vi "Initialization VI.vi"(8 "error in (no error)":errorcluster, 10 "Custom XML":string, 11 "Device Item Ref in":T1 format="%.0x") -> (0 "error out":errorcluster, 3 "Device Item Ref out":T1 format="%.0x")   [LabVIEW 2020, in "FPGA Addon System Explorer.lvlib"]
uses:
  FPGA Addon System Explorer.lvlib
  <vilib>/NI VeriStand/Custom Device API/Custom Device Item Ref.ctl
  Addon Shared/Types/FG Action.ctl
  Addon Shared/Types/FPGA Settings.ctl
  Addon Shared/SubVIs/Constants.vi
  <vilib>/NI VeriStand/Custom Device API/NI VeriStand - Get Item Property.vi
  <vilib>/NI VeriStand/Custom Device API/Get Item Property (Path).vi
  <vilib>/NI VeriStand/Custom Device API/Get Item Property (String).vi
  <vilib>/NI VeriStand/Custom Device API/Get Item Property (Boolean).vi
  <vilib>/NI VeriStand/Custom Device API/NI VeriStand - Set Item Property.vi
  <vilib>/NI VeriStand/Custom Device API/Set Item Property (Path).vi
  <vilib>/NI VeriStand/Custom Device API/Set Item Property (String).vi
  <vilib>/NI VeriStand/Custom Device API/Set Item Property (Boolean).vi
  <vilib>/NI/NI VeriStand Custom Device Import and Export Tool/ImportExport.lvlib
  Addon Shared/FPGA Addon Shared.lvlib
  <vilib>/NI VeriStand/Custom Device API/Custom Device API.lvlib
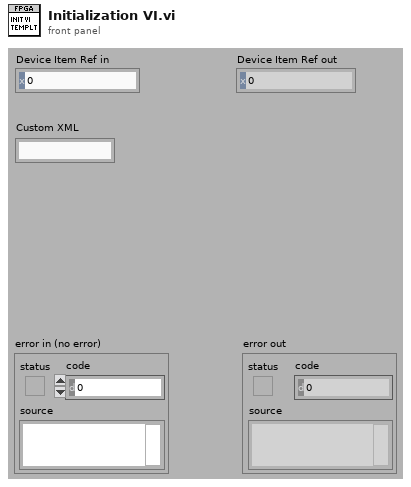
[diagram p1: front panel]
types:
  T1 = typedef "Custom Device API.lvlib/Custom Device Item Ref.ctl" = u64
  T2 = typedef "FPGA Addon Shared.lvlib/FPGA Settings.ctl" = cluster{"Bitfile path":path, "RIO Device Address":string, "Group":bool}
  T3 = typedef "FPGA Addon Shared.lvlib/FG Action.ctl" = enum8{"GET", "SET"}
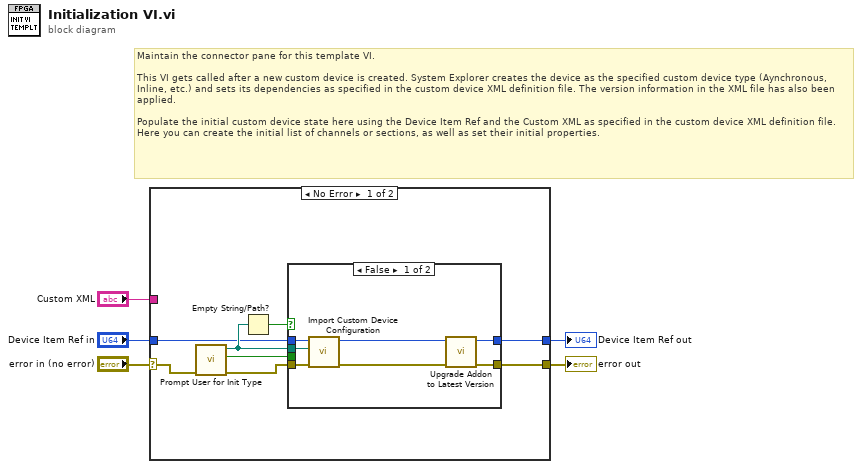
[diagram p0: block diagram]
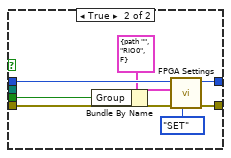
[diagram p2: hidden frame]
diagram:
  # "Maintain the connector pane for this template VI.\n\nThis VI gets called after a new custom device is created. System Explorer creates the device as the specified custom device type (Aynchronous, Inline, etc.) and sets its dependencies as specified in the custom device XML definition file. The version information in the XML file has also been applied.\n\nPopulate the initial custom device state here using the Device Item Ref and the Custom XML as specified in the custom device XML definition file. Here you can create the initial list of channels or sections, as well as set their initial properties."
  n1 = case shown="No Error" "error in (no error)" {
    selector: "error in (no error)" -> [w13 w30]
    tunnel: [w10 w30] -> w5
    tunnel: [w8 w29] -> w3
    tunnel: "Device Item Ref in" -> [w7 w29]
    tunnel: "Custom XML" -> [_ _]
    frame No Error {
      n2 = call "Prompt User for Init Type.vi"("error in (no error)"=w13) -> ("error out"=w11:errorcluster, "Group? out"=w6:bool, "Path out"=w9:path)  [unwired: 8 in]
      n3 = Empty String/Path?(string/path=w9) -> (empty?=w12:bool)
      n4 = case shown="False" w12 {
        tunnel: w11 -> [w18 w24]
        tunnel: [w17 w25] -> w10
        tunnel: w9 -> [w16 _]
        tunnel: w7 -> [w15 w27]
        tunnel: [w14 w26] -> w8
        tunnel: w6 -> [_ w21]
        frame False {
          n5 = call <vilib>:"Import Custom Device Configuration.vi"("error in (no error)"=w18, "Path"=w16, "NodeID"=w15) -> ("error out"=w20:errorcluster, "NodeID out"=w19:u64)  [unwired: 6 in, 1 out]
          n6 = call "Upgrade Addon to Latest Version.vi"("error in (no error)"=w20, "Device Item Ref in in"=w19) -> ("error out"=w17:errorcluster, "Device Item Ref out"=w14:T1)  [unwired: 8 in]
        }
        frame True {
          n7 = Bundle By Name(cluster=T2 {"Bitfile path"=path "", "RIO Device Address"="RIO0", "Group"=FALSE} ("FPGA Settings"), "Group"=w21) -> (w22:T2)
          n8 = call "FPGA Settings.vi"("Action"=FG_Action."SET", "error in (no error)"=w24, "FPGA Settings"=w22, "Item Ref"=w27) -> ("error out"=w25:errorcluster, "Item Ref out"=w26:T1)  [unwired: 5 in, 1 out]
        }
      }
    }
    frame Error {
    }
  }
  "error out" <- w5
  "Device Item Ref out" <- w3
